vi "Query.vi"(8 "error in (no error)":errorcluster, 9 "Prefix":string, 10 "command":string="command", 11 "VISA resource name":refnum<visa-resource-name>) -> (0 "error out":errorcluster, 2 "Reply":string, 3 "VISA Res OUT":refnum<visa-resource-name>)   [LabVIEW 2026]
uses:
  <vilib>/Utility/error.llb/Trim Whitespace (string).vi
  <vilib>/Utility/error.llb/Trim Whitespace One-Sided.vi
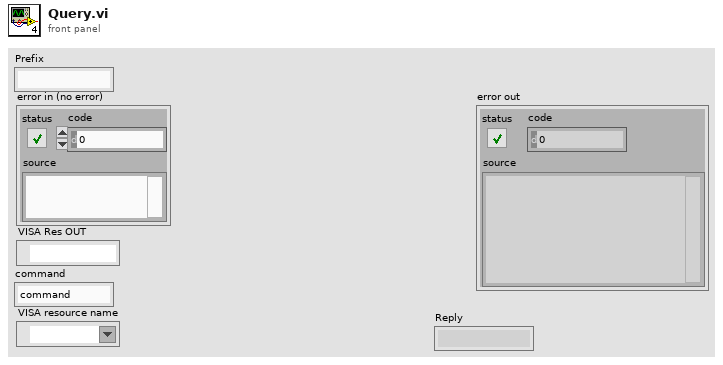
[diagram p1: front panel]
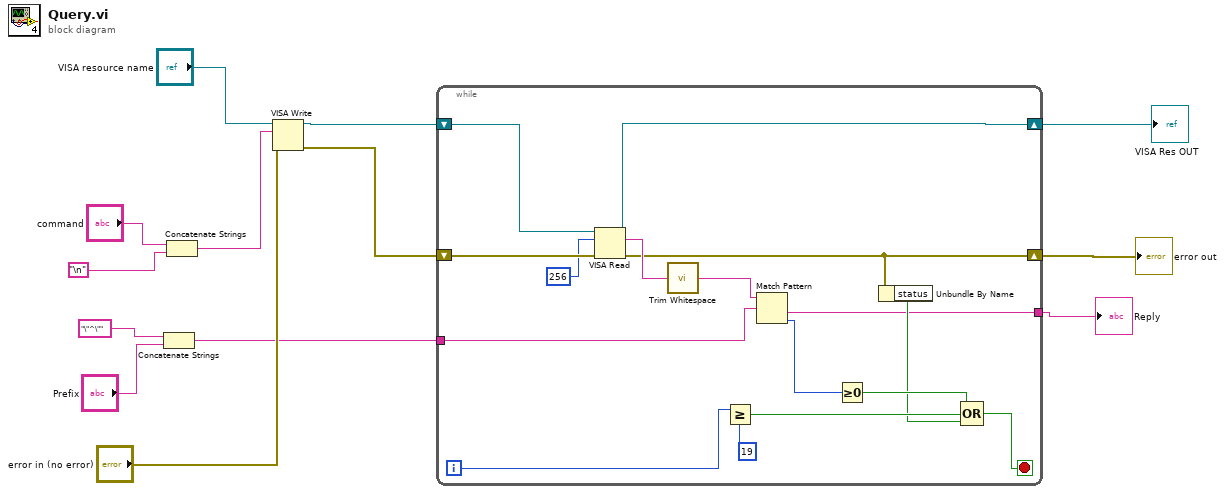
[diagram p0: block diagram]
diagram:
  n1 = Concatenate Strings("\"^\"" ("string"), "Prefix") -> (w6:string)
  n2 = Concatenate Strings("command", "\n") -> (w5:string)
  n3 = VISA Write(VISA resource name="VISA resource name", write buffer=w5, error in (no error)="error in (no error)") -> (VISA resource name out=w8:refnum<visa-resource-name>, error out=w7:errorcluster)  [unwired: 1 out]
  n4 = while {
    shift-right: [w18] -> w4
    shift-left: w8 -> [w27]
    shift-right: [w16] -> w3
    shift-left: w7 -> [w26]
    tunnel: w6 -> [w25]
    tunnel: [w14] -> w2
    i -> [w21]
    stop <- w17 stop-if-true
    n5 = VISA Read(VISA resource name=w27, byte count=u32 256, error in (no error)=w26) -> (VISA resource name out=w18:refnum<visa-resource-name>, read buffer=w29:string, error out=w16:errorcluster)  [unwired: 1 out]
    n6 = call-poly <vilib>:"Trim Whitespace.vi"("string"=w29) -> ("trimmed string"=w28:string)  [unwired: 1 in]
    n7 = Greater Or Equal?(x=w21, y=19) -> (x >= y?=w19:bool)
    n8 = Match Pattern(string=w28, regular expression=w25) -> (after substring=w14:string, offset past match=w23:i32)  [unwired: 1 in, 2 out]
    n9 = Greater Or Equal To 0?(x=w23) -> (x >= 0?=w22:bool)
    n10 = Unbundle By Name(w16) -> ("status"=w15:bool)
    n11 = Compound Arithmetic op=OR(w22, w19, w15) -> (w17:bool)
  }
  "VISA Res OUT" <- w4
  "error out" <- w3
  "Reply" <- w2
